vi "Buffer_GPIB_SR400.vi"(11 "N per point":i32=1) -> (1 "Array":string[](array[string]), 2 "x/y":dbl)   [LabVIEW 2025]
uses:
  <vilib>/Utility/error.llb/Trim Whitespace One-Sided.vi
  GPIB_Address.vi
panel:
  in  "VISA resource name":refnum<visa-resource-name>="GPIB0::23::INSTR"
  out "String":string
  out "output array":string[](array[string])
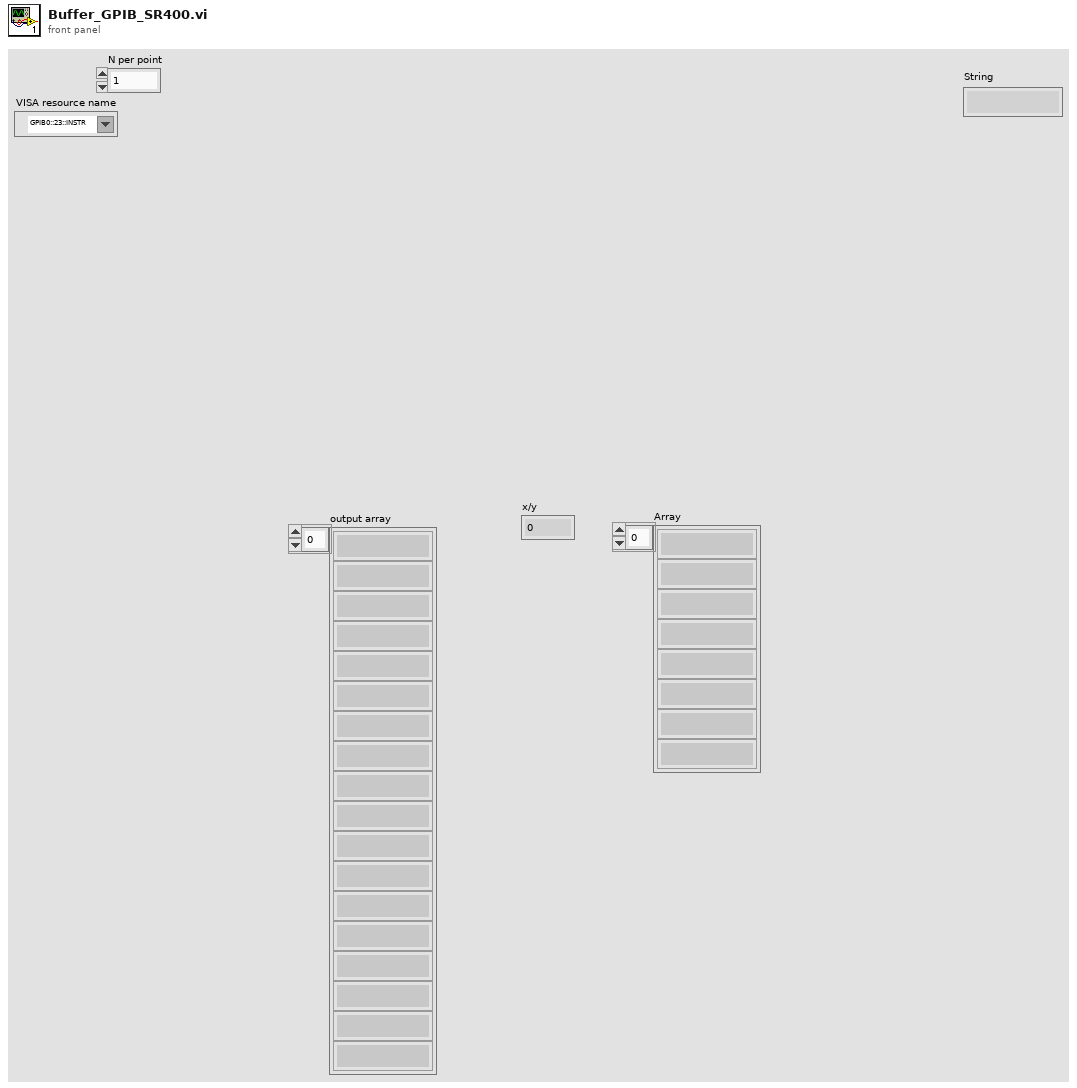
[diagram p1: front panel]
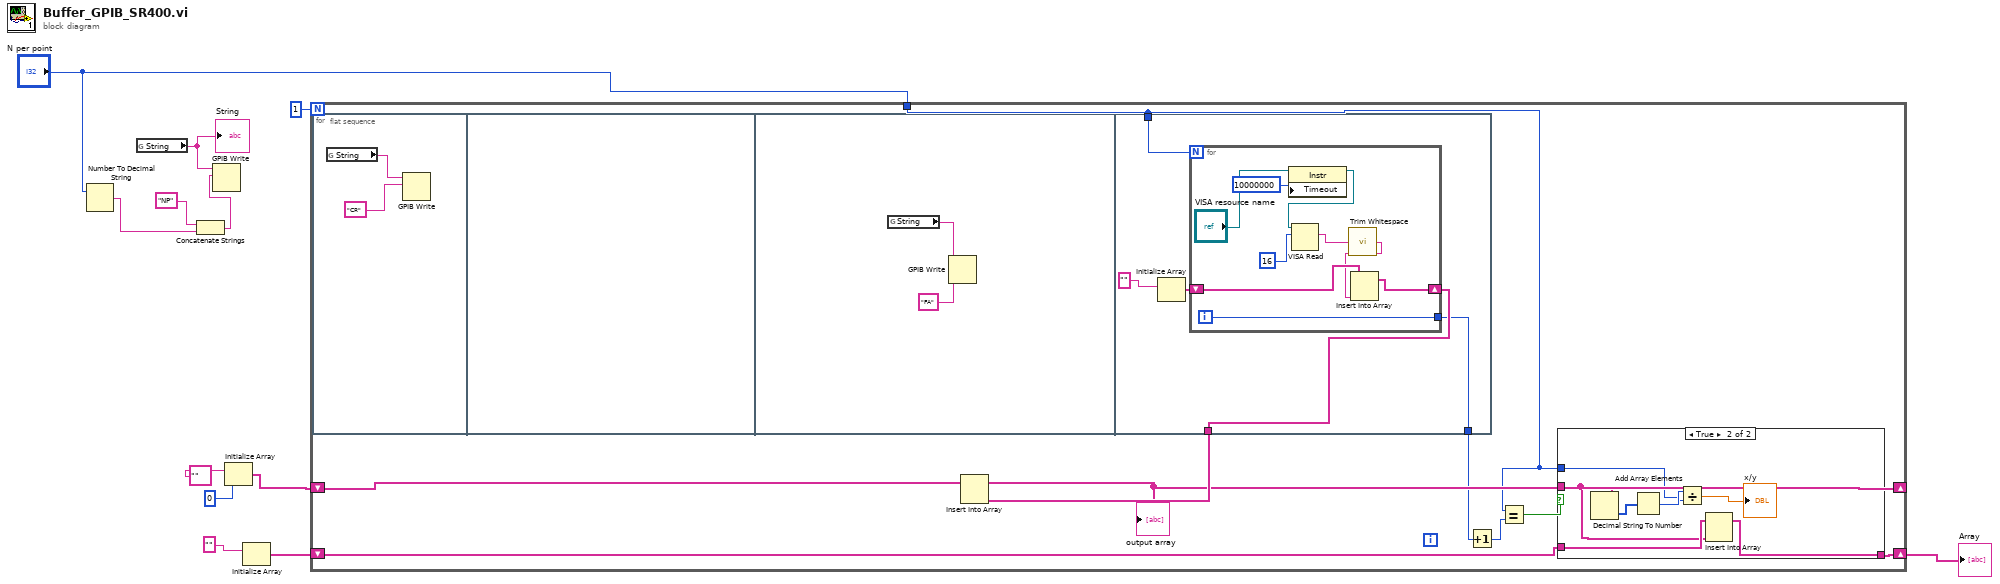
[diagram p0: block diagram]
diagram:
  n1 = Number To Decimal String(number="N per point") -> (decimal integer string=w2:string)  [unwired: 1 in]
  n2 = global read "GPIB_Address.vi" "String"() -> (w5:string)
  "String" <- w5
  n3 = Concatenate Strings("NP" ("data"), w2) -> (w1:string)
  n4 = GPIB Write(0:w5, 1:w1) -> ()  [unwired: 3 in, 2 out]
  n5 = Initialize Array("", 0 ("dimension size")) -> (w11:string[])
  n6 = Initialize Array("") -> (w8:string[])  [unwired: 1 in]
  n7 = for {
    N: 1 -> [_]
    shift-right: [w18] -> _
    shift-left: w11 -> [w21]
    shift-right: [w16] -> w7
    shift-left: w8 -> [w15]
    tunnel: "N per point" -> [w14]
    n8 = flat-sequence {
      tunnel: [w34] -> w20
      tunnel: w14 -> [w37]
      tunnel: [w33] -> w13
      frame #0 {
        n9 = global read "GPIB_Address.vi" "String"() -> (w29:string)
        n10 = GPIB Write(0:w29, 1:"CR" ("data")) -> ()  [unwired: 3 in, 2 out]
      }
      frame #1 {
      }
      frame #2 {
        n11 = global read "GPIB_Address.vi" "String"() -> (w31:string)
        n12 = GPIB Write(0:w31, 1:"FA" ("data")) -> ()  [unwired: 3 in, 2 out]
      }
      frame #3 {
        n13 = Initialize Array("") -> (w35:string[])  [unwired: 1 in]
        n14 = for {
          N: w37 -> [_]
          shift-right: [w44] -> w34
          shift-left: w35 -> [w45]
          tunnel: [w38] -> w33
          i -> [w38]
          n15 = property class="Instr"(reference="VISA resource name", "Timeout"=u32 10000000 ("General Settings:Timeout Value")) -> (reference out=w39:refnum<visa-resource-name>)  [unwired: 1 in, 1 out]
          n16 = VISA Read(VISA resource name=w39, byte count=16) -> (read buffer=w42:string)  [unwired: 1 in, 3 out]
          n17 = call <vilib>:"Trim Whitespace.vi"("string"=w42) -> ("trimmed string"=w43:string)  [unwired: 1 in]
          n18 = Insert Into Array "Insert Into Array"(array=w45, new element=w43) -> (w44:string[])  [unwired: 1 in]
        }
      }
    }
    n19 = Insert Into Array "Insert Into Array"(array=w21, new element=w20) -> (w18:string[])  [unwired: 1 in]
    "output array" <- w18
    n20 = Increment(x=w13) -> (x+1=w17:i32)
    n21 = Equal?(x=w14, y=w17) -> (x = y?=w19:bool)
    n22 = case shown="True" w19 {
      tunnel: w18 -> [_ w23]
      tunnel: w14 -> [_ w26]
      tunnel: [_ w22] -> w16
      tunnel: w15 -> [_ w24]
      frame False {
      }
      frame True {
        n23 = Decimal String To Number(string=w23) -> (number=w28:i32[])  [unwired: 2 in, 1 out]
        n24 = Add Array Elements(numeric array=w28) -> (sum=w27:i32)
        n25 = Divide(x=w27, y=w26) -> (x/y=→"x/y":dbl)
        n26 = Insert Into Array(array=w24, new element=w23) -> (w22:string[])  [unwired: 1 in]
      }
    }
  }
  "Array" <- w7
